vi "SMTP Email Send Multiple Attachments Message.vi"(0 "smtp session":T1 caption="session smtp", 1 "attachments":T2(array[cluster]) caption="pièces jointes", 2 "return address":string caption="adresse de retour", 3 "character set":string caption="jeu de caractères", 5 "recipients":string[](array[string]) caption="destinataires", 7 "subject":string caption="objet", 9 "message":string, 11 "error in (no error)":errorcluster caption="entrée d'erreur (pas d'erreur)", 12 "translit":string="MacRoman iso-8859-1 macroman.trl, ToUpper iso-8859-1 toupper.trl,\nMacRomanUp MacRoman toupper.trl") -> (4 "smtp session out":T1 caption="session smtp en sortie", 6 "invalid recipients":string[](array[string]) caption="destinataires non valides", 15 "error out":errorcluster caption="sortie d'erreur")   [LabVIEW 2022 SP3, in "Copie de NI_SMTPEmail.lvlib"]
doc: "Envoie par e-mail le message textuel et les pièces jointes vers les destinataires en utilisant Mailserver.\n\nMessage textuel : message textuel à envoyer ; s'il n'y en a pas, seules les pièces jointes seront envoyées.\n\nPièces jointes : tableau de clusters contenant quatre champs : 1) S'il s'agit d'un fichier ou de données enregistrées ; 2) Si ce sont des données enregistrées, ces données apparaissent dans le champ ; sinon le nom du fichier où récupérer les données doit être câblé ici ; 3) Si les données sont-elles binaires ou textuelles ; 4) Si les données sont binaires, de quel type sont-elles (cad application/octet-stream (par défaut), image/jpeg, image/gif, etc.)\n\nMailserver : serveur de messagerie SMTP à utiliser pour envoyer l'e-mail. Doit être spécifié ici ou configuré en utilisant SMTP Setup.vi\n\nAdresse de retour : l'adresse de retour de votre choix ; elle peut être spécifiée ici ou configurée en utilisant SMTP Setup.vi\n\nDestinataires : liste des adresses e-mail vers où envoyer votre e-mail.\n\nObjet : objet de votre message. \"Aucune\" est la chaîne par défaut si l'entrée n'est pas câblée.\n\nJeu de caractères : la messagerie fournit un support international. La valeur de jeu de caractères est nécessaire pour fonctionner avec les jeux de caractères étrangers (non-US).\n\nDestinataires non valides : la liste des destinataires (hormis ceux spécifiés) qui n'existent pas selon le serveur mail (qui peut très bien ne pas contenir tous les destinataires non valides, surtout s'ils ne sont pas locaux pour le serveur SMTP)."
uses:
  Copie de NI_SMTPEmail.lvlib
  SMTP Email Session.ctl
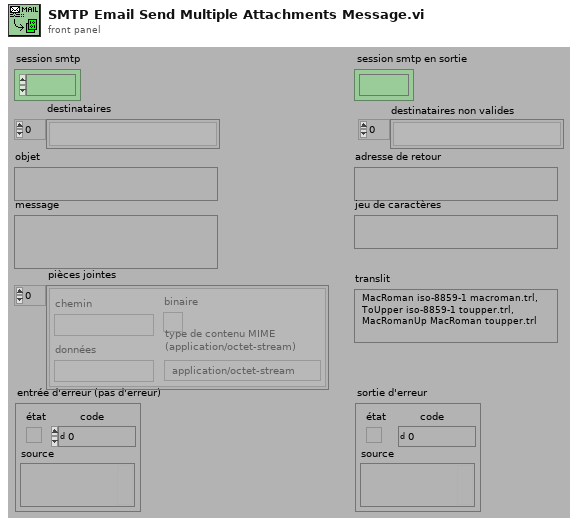
[diagram p1: front panel]
types:
  T1 = typedef "Copie de NI_SMTPEmail.lvlib/SMTP Email Session.ctl" = refnum<k1>
  T2 = cluster{"path":path, "data":string, "binary":bool, "MIME content-type \n(application/octet-stream)":string}[]
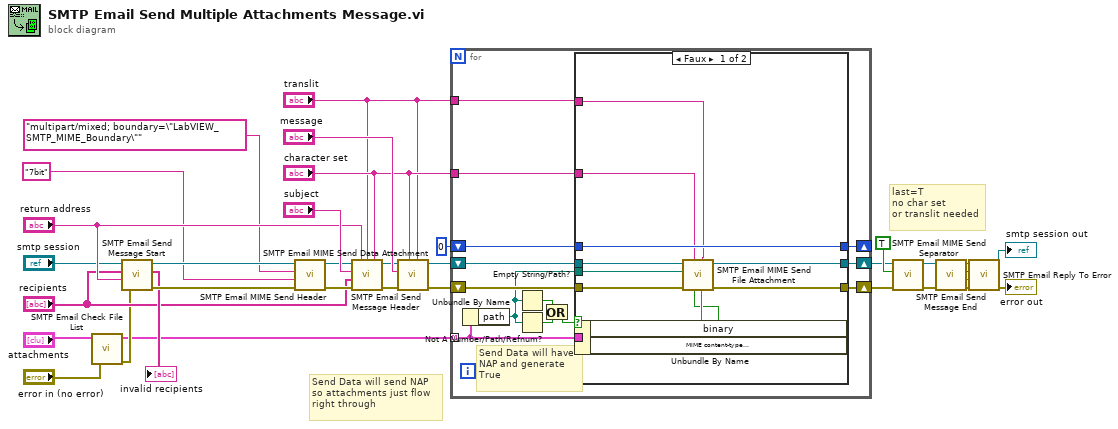
[diagram p0: block diagram]
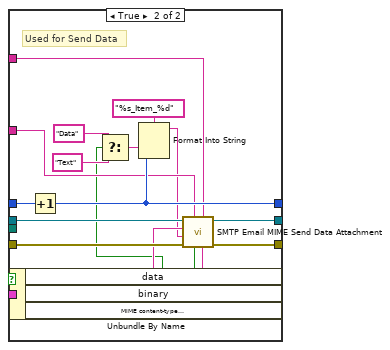
[diagram p2: hidden frame]
diagram:
  # "Send Data will send NAP\nso attachments just flow\nright through"
  # "last=T\nno char set\nor translit needed"
  n1 = call "SMTP Email Check File List.vi"("error in (no error)"="error in (no error)", "attachments"="attachments") -> ("error out"=w14:errorcluster, "attachments out"=w11:T2)  [unwired: 4 in]
  n2 = call "SMTP Email Send Message Start.vi"("error in (no error)"=w14, "return address"="return address", "recipients"="recipients", "smtp session"="smtp session") -> ("error out"=w20:errorcluster, "invalid recipients"=→"invalid recipients":string[], "smtp session out"=w21:T1)  [unwired: 1 in]
  n3 = call "SMTP Email MIME Send Header.vi"("error in (no error)"=w20, "MIME content-transfer-encoding (7bit)"="7bit", "MIME content-type (multipart/mixed)"="multipart/mixed; boundary=\"LabVIEW_SMTP_MIME_Boundary\"", "smtp session"=w21) -> ("error out"=w25:errorcluster, "smtp session out"=w26:T1)  [unwired: 2 in]
  n4 = call "SMTP Email Send Message Header.vi"("character set"="character set", "translit"="translit", "return address"="return address", "error in (no error)"=w25, "recipients"="recipients", "subject"="subject", "smtp session"=w26) -> ("error out"=w28:errorcluster, "smtp session out"=w27:T1)  [unwired: 3 in]
  n5 = call "SMTP Email MIME Send Data Attachment.vi"("translit"="translit", "character set"="character set", "error in (no error)"=w28, "data"="message", "smtp session"=w27) -> ("error out"=w22:errorcluster, "smtp session out"=w23:T1)  [unwired: 5 in]
  n6 = for {
    tunnel: w11 -> [w47] mode=indexing
    shift-right: [w45] -> w29
    shift-left: w23 -> [w46]
    shift-right: [w41] -> w30
    shift-left: w22 -> [w42]
    shift-right: [w43] -> _
    shift-left: 0 -> [w44]
    tunnel: "character set" -> [w40]
    tunnel: "translit" -> [w35]
    # "Send Data will have\nNAP and generate\nTrue"
    n7 = Unbundle By Name(w47) -> ("path"=w39:path)
    n8 = Empty String/Path?(string/path=w39) -> (empty?=w37:bool)
    n9 = Not A Number/Path/Refnum?(number/path/refnum=w39) -> (NaN/Path/Refnum?=w38:bool)
    n10 = Or(x=w37, y=w38) -> (x .or. y?=w36:bool)
    n11 = case shown="Faux" w36 {
      tunnel: [w55 w70] -> w45
      tunnel: [w54 w71] -> w41
      tunnel: w46 -> [w56 w73]
      tunnel: w42 -> [w57 w72]
      tunnel: w44 -> [w58 w67]
      tunnel: [w58 w65] -> w43
      tunnel: w39 -> [w53 _]
      tunnel: w47 -> [w50 w74]
      tunnel: w40 -> [w49 w62]
      tunnel: w35 -> [w48 w59]
      frame False {
        n12 = Unbundle By Name(w50) -> ("binary"=w51:bool, "MIME content-type \n(application/octet-stream)"=w52:string)
        n13 = call "SMTP Email MIME Send File Attachment.vi"("MIME content-type"=w52, "translit"=w48, "binary (F)"=w51, "character set"=w49, "error in (no error)"=w57, "path"=w53, "smtp session"=w56) -> ("error out"=w54:errorcluster, "smtp session out"=w55:T1)  [unwired: 2 in, 1 out]
      }
      frame True {
        # "Used for Send Data"
        n14 = Unbundle By Name(w74) -> ("data"=w64:string, "binary"=w60:bool, "MIME content-type \n(application/octet-stream)"=w63:string)
        n15 = Increment(x=w67) -> (x+1=w65:i32)
        n16 = Select(t="Data", s=w60, f="Text") -> (s? t:f=w68:string)
        n17 = Format Into String(format string="%s_Item_%d", w68, w65) -> (resulting string=w61:string)  [unwired: 2 in, 1 out]
        n18 = call "SMTP Email MIME Send Data Attachment.vi"("MIME content-type"=w63, "translit"=w59, "binary (F)"=w60, "character set"=w62, "error in (no error)"=w72, "name"=w61, "data"=w64, "smtp session"=w73) -> ("error out"=w71:errorcluster, "smtp session out"=w70:T1)  [unwired: 2 in]
      }
    }
  }
  n19 = call "SMTP Email MIME Send Separator.vi"("error in (no error)"=w30, "last (F)"=TRUE, "smtp session"=w29) -> ("error out"=w17:errorcluster, "smtp session out"=w16:T1)  [unwired: 7 in]
  n20 = call "SMTP Email Send Message End.vi"("error in (no error)"=w17, "smtp session"=w16) -> ("error out"=w10:errorcluster, "reply"=w5:string, "reply code"=w6:i32, "smtp session out"=w9:T1)  [unwired: 2 in]
  n21 = call "SMTP Email Reply To Error.vi"("error in (no error)"=w10, "reply string in"=w5, "reply code in"=w6, "smtp session"=w9) -> ("error out"=→"error out":errorcluster, "smtp session out"=→"smtp session out":T1)  [unwired: 2 out]
